vi "Open Session SFTP.vi"(6 "Timeout(ms)":i32=5000, 7 "TargetIP":string, 8 "error in (no error)":errorcluster, 10 "Password":string, 11 "Username":string) -> (0 "error out":errorcluster, 3 "SFTP session":refnum<class "Session.lvclass">)   [LabVIEW 2027, in "VeriStandTestUtilities.lvlib"]
uses:
  <vilib>/net/SFTP/Session/Session.lvclass
  <vilib>/net/SSH/Client/OpenSSH/OpenSSH Client.lvclass
  <vilib>/net/SSH/Client/Generic/Generic Client.lvclass/Generic Client.ctl
  <vilib>/net/SSH/Client/Generic/Write trust on first use.vi
  <vilib>/net/SFTP/Connect (OpenSSH).vi
  VeriStandTestUtilities.lvlib
  <vilib>/net/SFTP/NI_SFTP.lvlib
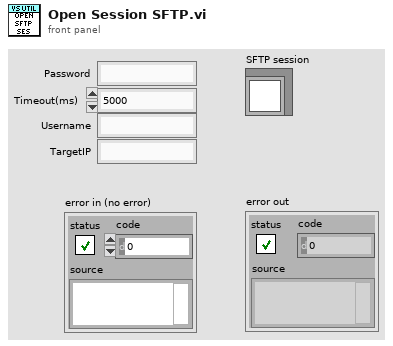
[diagram p1: front panel]
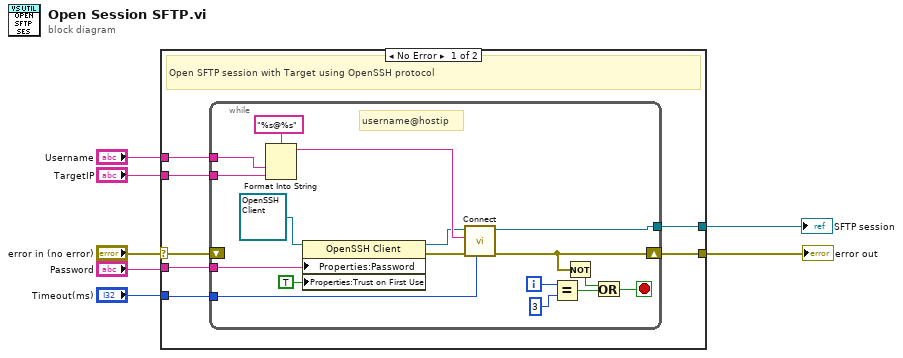
[diagram p0: block diagram]
diagram:
  n1 = case shown="No Error" "error in (no error)" {
    selector: "error in (no error)" -> [w14 w32]
    tunnel: [w10 w32] -> w6
    tunnel: "Timeout(ms)" -> [w9 _]
    tunnel: "Password" -> [w13 _]
    tunnel: "Username" -> [w12 _]
    tunnel: "TargetIP" -> [w11 _]
    tunnel: [w8 _] -> w1
    frame No Error {
      # "Open SFTP session with Target using OpenSSH protocol"
      n2 = while {
        tunnel: w13 -> [w30]
        tunnel: w12 -> [w26]
        tunnel: w11 -> [w25]
        tunnel: w9 -> [w22]
        tunnel: [w21] -> w8
        shift-right: [w16] -> w10
        shift-left: w14 -> [_]
        i -> [w20]
        stop <- w15 stop-if-true
        # "username@hostip"
        n3 = Format Into String(format string="%s@%s", w26, w25) -> (resulting string=w24:string)  [unwired: 2 in, 1 out]
        n4 = property class="OpenSSH Client"(reference=refnum<class "OpenSSH Client.lvclass"> refnum ("client"), "Properties:Password"=w30, "Properties:Trust on First Use"=TRUE ("trust on first use")) -> (reference out=w23:refnum<class "OpenSSH Client.lvclass">, error out=w29:errorcluster)  [unwired: 1 in]
        n5 = call-poly <vilib>:"Connect.vi"("timeout (ms)"=w22, "error in"=w29, "user@host"=w24, "client"=w23) -> ("error out"=w16:errorcluster, "session"=w21:refnum<class "Session.lvclass">)  [unwired: 6 in]
        n6 = Equal?(x=w20, y=3) -> (x = y?=w18:bool)
        n7 = Not(x=w16) -> (.not. x?=w17:bool)
        n8 = Or(x=w17, y=w18) -> (x .or. y?=w15:bool)
      }
    }
    frame Error {
    }
  }
  "error out" <- w6
  "SFTP session" <- w1
